vi "1.3.vi"() -> ()   [LabVIEW 2026]
panel:
  out "F":dbl(slide) scale=0.0..100.0
  in  "C":dbl(slide) scale=0.0..100.0
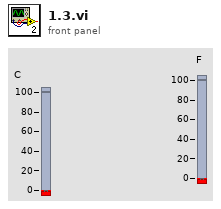
[diagram p1: front panel]
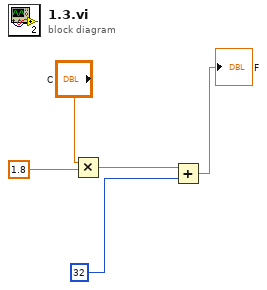
[diagram p0: block diagram]
diagram:
  n1 = Multiply(x="C", y=1.8) -> (x*y=w3:dbl)
  n2 = Add(x=w3, y=32) -> (x+y=→"F":dbl)
